vi "Exp - errno value.vi"(5 "InstanceRef":T1, 6 "error in":bool, 7 "action":enum32{"get", "set"}(ring), 9 "errno value":i32) -> (0 "error out":bool, 2 "prev errno value":i32, 3 "errno value out":i32)   [LabVIEW 2021]
doc: "::: CalcExpress Toolkit :::\nCopyright (c) 2000-2026 Konstantin Shifershteyn. All rights reserved."
uses:
  cetypes.llb/CalcExpress Instance RefNum.ctl
  cersrc/celveng32.dll
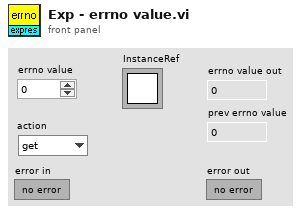
[diagram p1: front panel]
types:
  T1 = typedef "CalcExpress Instance RefNum.ctl" = refnum<k1>
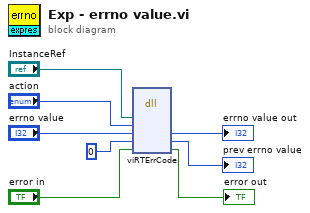
[diagram p0: block diagram]
diagram:
  n1 = dll-call lib="C:/LV Projects/CalcExpress 40 LV2021/vi.lib/addons/CalcExpress/cersrc/celveng*.dll" fn="viRTErrCode"("iRef"="InstanceRef", "cmd"="action", "errno"="errno value", "prev_errno"=0 ("errno value"), "erf"="error in") -> ("errno"=→"errno value out":i32, "prev_errno"=→"prev errno value":i32, "erf"=→"error out":bool)  [unwired: 6 in, 2 out]
